vi "RemoteVI Application Example.vi"() -> ()   [LabVIEW 2020]
doc: "This example demonstrates the use of splitter bars to divide the front panel into multiple panes. Each pane can be set up to behave differently depending on the desired function of each pane. In this example the graphical display contained in the lower right pane has the ability to resize with the pane."
uses:
  source/RemoteVI.lvlib
panel:
  out "error out":errorcluster
  in  "Menu":i32(listbox)
  in  "Quit":bool
  out "Remote Link":string
  out "Page":string
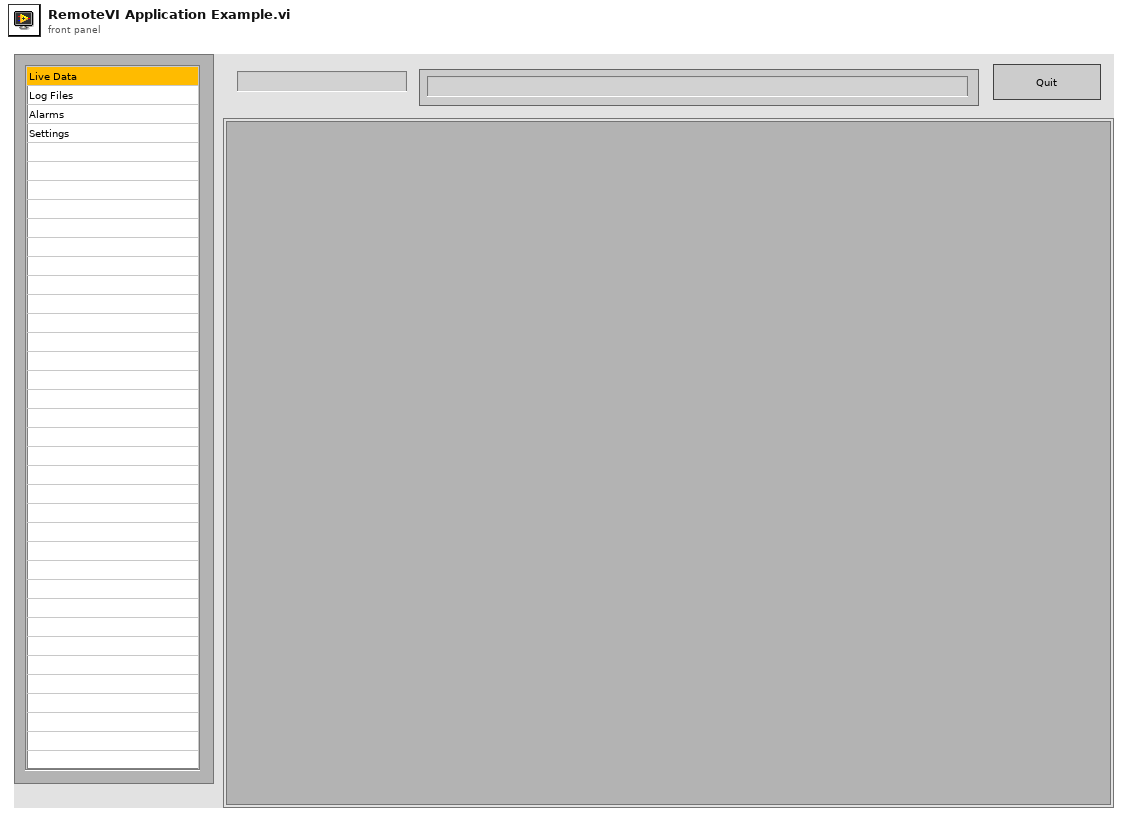
[diagram p1: front panel]
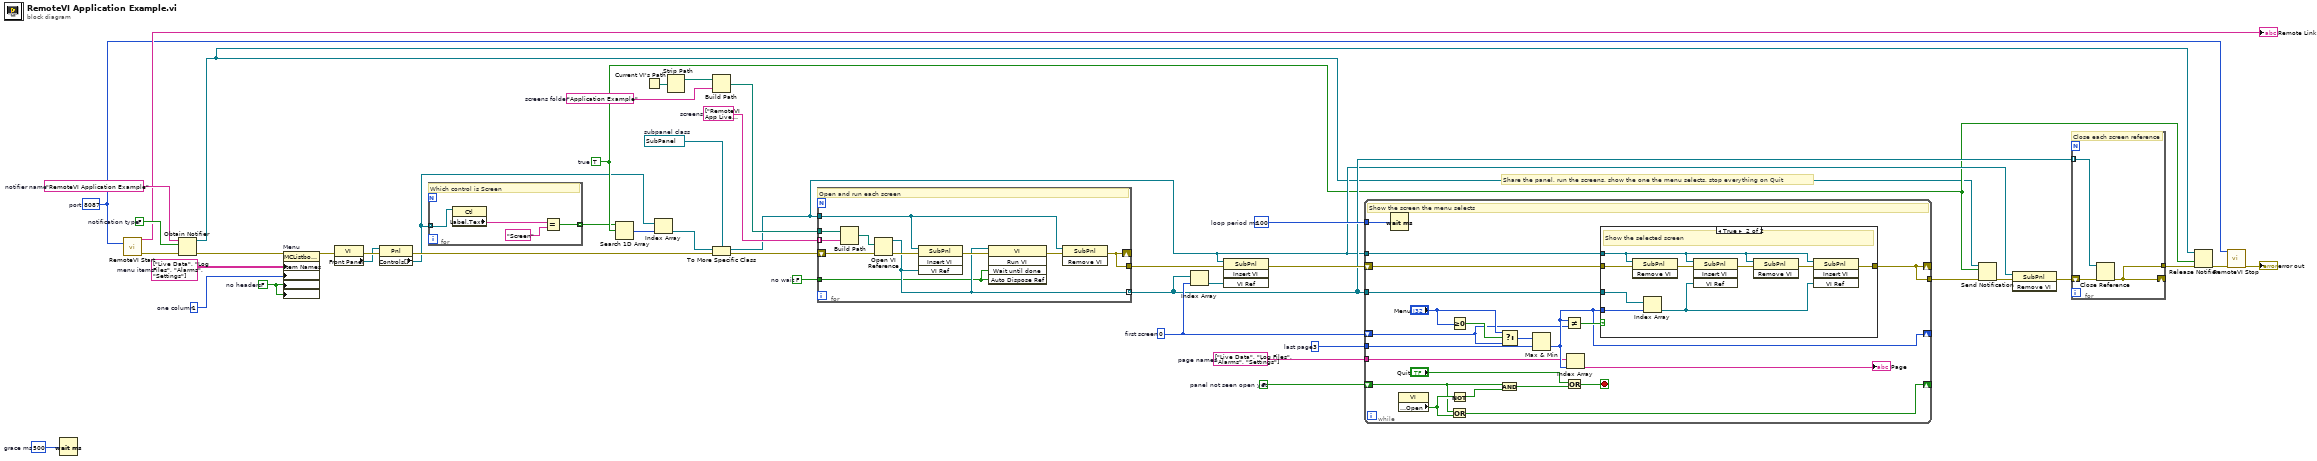
[diagram p0: block diagram]
diagram:
  w40 = 500  # grace ms
  w37 = FALSE  # panel not seen open yet
  w36 = 3  # last page
  w35 = 100  # loop period ms
  w34 = string[] ["Live Data", "Log Files", "Alarms", "Settings"]  # page names
  w31 = 0  # first screen
  w28 = FALSE  # no wait
  w27 = string[] ["RemoteVI App Live Data.vi", "RemoteVI App Log Files.vi", "RemoteVI App Alarms.vi", "RemoteVI App Settings.vi"]  # screens
  w25 = "Application Example"  # screens folder
  w20 = refnum<vi> refnum  # subpanel class
  w17 = TRUE  # true
  w10 = FALSE  # no headers
  w9 = 1  # one column
  w8 = string[][] [["Live Data"], ["Log Files"], ["Alarms"], ["Settings"]]  # menu items
  w5 = FALSE  # notification type
  w4 = "RemoteVI Application Example"  # notifier name
  w1 = u16 8087  # port
  # "Share the panel, run the screens, show the one the menu selects, stop everything on Quit"
  n1 = Wait (ms)(milliseconds to wait=w40) -> ()  [unwired: 1 out]
  n2 = call "RemoteVI Start.vi"("port"=w1) -> ("URL"=→"Remote Link":string, "error out"=w3:errorcluster)  [unwired: 13 in]
  n3 = Obtain Notifier(name (unnamed)=w4, notification data type=w5, error in (no error)=w3) -> (notifier out=w6:refnum<notifier>, error out=w7:errorcluster)  [unwired: 1 in, 1 out]
  n4 = property on="Menu" class="MCListbox (strict)"(error in=w7, "Item Names"=w8, "Number of Columns"=w9, "Visible Items:Column Headers Visible"=w10, "Visible Items:Horizontal Scrollbar Visible"=w10) -> (error out=w11:errorcluster)  [unwired: 1 in, 1 out]
  n5 = property class="VI"(error in=w11) -> (error out=w13:errorcluster, "Front Panel"=w12:refnum<vi>)  [unwired: 1 in, 1 out]
  n6 = property class="Pnl"(reference=w12, error in=w13) -> (error out=w15:errorcluster, "Controls[]"=w14:refnum<vi>[])  [unwired: 1 out]
  n7 = for {
    tunnel: w14 -> [w45] mode=indexing
    tunnel: [w48] -> w16 mode=indexing
    # "Which control is Screen"
    n8 = property class="Ctl"(reference=w45) -> ("Label.Text"=w46:string)  [unwired: 1 in, 2 out]
    n9 = Equal?(x=w46, y="Screen") -> (x = y?=w48:bool)
  }
  n10 = Search 1D Array(1D array=w16, element=w17) -> (index of element=w18:i32)  [unwired: 1 in]
  n11 = Current VI's Path() -> (path=w23:path)
  n12 = Index Array(array=w14, index=w18) -> (element=w19:refnum<vi>)
  n13 = Strip Path(path=w23) -> (stripped path=w24:path)  [unwired: 1 out]
  n14 = Build Path(base path=w24, name or relative path=w25) -> (appended path=w26:path)
  n15 = To More Specific Class(target class=w20, reference=w19, error in=w15) -> (specific class reference=w21:refnum<vi>, error out=w22:errorcluster)
  n16 = for {
    tunnel: w27 -> [w49] mode=indexing
    tunnel: w28 -> [w51]
    tunnel: w26 -> [w50]
    tunnel: w21 -> [w52]
    shift-right: [w54] -> _
    shift-left: w22 -> [w53]
    tunnel: [w56] -> w29 mode=indexing
    tunnel: [w54] -> w30
    # "Open and run each screen"
    n17 = Build Path(base path=w50, name or relative path=w49) -> (appended path=w55:path)
    n18 = Open VI Reference(vi path=w55, error in (no error)=w53) -> (vi reference=w56:refnum<vi>, error out=w57:errorcluster)  [unwired: 4 in]
    n19 = invoke class="SubPnl" method="Insert VI"(reference=w52, error in=w57, "VI Ref"=w56) -> (error out=w58:errorcluster)  [unwired: 1 in, 3 out]
    n20 = invoke class="VI" method="Run VI"(reference=w56, error in=w58, "Wait until done"=w51, "Auto Dispose Ref"=w51) -> (error out=w59:errorcluster)  [unwired: 1 in, 4 out]
    n21 = invoke class="SubPnl" method="Remove VI"(reference=w52, error in=w59) -> (error out=w54:errorcluster)  [unwired: 1 in, 2 out]
  }
  n22 = Index Array(array=w29, index=w31) -> (element=w32:refnum<vi>)
  n23 = invoke class="SubPnl" method="Insert VI"(reference=w21, error in=w30, "VI Ref"=w32) -> (error out=w33:errorcluster)  [unwired: 1 in, 3 out]
  n24 = while {
    tunnel: w34 -> [w62]
    tunnel: w35 -> [w63]
    tunnel: w36 -> [w64]
    shift-right: [w66] -> _
    shift-left: w31 -> [w65]
    shift-right: [w70] -> _
    shift-left: w37 -> [w69]
    tunnel: w21 -> [w60]
    tunnel: w29 -> [w61]
    shift-right: [w68] -> _
    shift-left: w33 -> [w67]
    tunnel: [w68] -> w38
    stop <- w80 stop-if-true
    # "Show the screen the menu selects"
    n25 = Wait (ms)(milliseconds to wait=w63) -> ()  [unwired: 1 out]
    n26 = property class="VI"() -> ("Front Panel Window:Open"=w77:bool)  [unwired: 2 in, 2 out]
    n27 = Greater Or Equal To 0?(x="Menu") -> (x >= 0?=w73:bool)
    n28 = Not(x=w77) -> (.not. x?=w78:bool)
    n29 = Or(x=w69, y=w77) -> (x .or. y?=w70:bool)
    n30 = And(x=w69, y=w78) -> (x .and. y?=w79:bool)
    n31 = Select(t="Menu", s=w73, f=w65) -> (s? t:f=w74:i32)
    n32 = Max & Min(x=w74, y=w64) -> (min(x,y)=w66:i32)  [unwired: 1 out]
    n33 = Not Equal?(x=w66, y=w65) -> (x != y?=w75:bool)
    n34 = Or(x="Quit", y=w79) -> (x .or. y?=w80:bool)
    n35 = Index Array(array=w62, index=w66) -> (element=→"Page":string)
    n36 = case shown="True" w75 {
      tunnel: w66 -> [_ w84]
      tunnel: w60 -> [_ w82]
      tunnel: w61 -> [_ w83]
      tunnel: w67 -> [w81 w85]
      tunnel: [w81 w90] -> w68
      frame False {
        # "Same screen"
      }
      frame True {
        # "Show the selected screen"
        n37 = invoke class="SubPnl" method="Remove VI"(reference=w82, error in=w85) -> (error out=w86:errorcluster)  [unwired: 1 in, 2 out]
        n38 = Index Array(array=w83, index=w84) -> (element=w87:refnum<vi>)
        n39 = invoke class="SubPnl" method="Insert VI"(reference=w82, error in=w86, "VI Ref"=w87) -> (error out=w88:errorcluster)  [unwired: 1 in, 3 out]
        n40 = invoke class="SubPnl" method="Remove VI"(reference=w82, error in=w88) -> (error out=w89:errorcluster)  [unwired: 1 in, 2 out]
        n41 = invoke class="SubPnl" method="Insert VI"(reference=w82, error in=w89, "VI Ref"=w87) -> (error out=w90:errorcluster)  [unwired: 1 in, 3 out]
      }
    }
  }
  n42 = Send Notification(notification=w17, notifier=w6, error in (no error)=w38) -> (error out=w39:errorcluster)  [unwired: 1 out]
  n43 = invoke class="SubPnl" method="Remove VI"(reference=w21, error in=w39) -> (error out=w41:errorcluster)  [unwired: 1 in, 2 out]
  n44 = for {
    tunnel: w29 -> [w91] mode=indexing
    shift-right: [w93] -> _
    shift-left: w41 -> [w92]
    tunnel: [w93] -> w42
    # "Close each screen reference"
    n45 = Close Reference(reference=w91, error in (no error)=w92) -> (error out=w93:errorcluster)
  }
  n46 = Release Notifier(notifier=w6, force destroy? (F)=w17, error in (no error)=w42) -> (error out=w43:errorcluster)  [unwired: 2 out]
  n47 = call "RemoteVI Stop.vi"("port"=w1, "error in"=w43) -> ("error out"=→"error out":errorcluster)  [unwired: 13 in]
